vi "REV Sequence.vi"() -> ()   [LabVIEW 2026]
uses:
  <vilib>/REVLibDriver5/subvi/RevLibError.ctl
  <vilib>/REV Custom Controls/c_Spark_SparkModel.ctl
  <vilib>/REV Custom Controls/c_Spark_MotorType.ctl
  <vilib>/REV Custom Controls/c_Spark_ConfigParameter.ctl
  <vilib>/REV Custom Controls/c_Spark_ControlType.ctl
  236934de-075f-3feb-e829-b4f31b15ce3f.vi
  <vilib>/REVLibDriver5/REVLibDriver.lvlib
  lib/libREVLibDriver.so
  lvaddons/wpilib/1/MrcLib.lvlib
panel:
  out "function return 7":T1
  in  "Slide":dbl(slide) scale=-1.0..1.0
  out "function return 6":T1
  out "value out":u8
  out "function return 5":T1
  in  "idle":bool
  out "c_Spark_SparkModel":T2 items=["c_Spark_Unknown", "c_Spark_SparkFlex", "c_Spark_SparkMax"]
  out "function return 4":T1
  out "fwVersion out":T3
  in  "stop":bool
  out "function return 3":T1
  out "function return 2":T1
  out "function return":T1
  out "deviceId out":i32
  out "status out":T1
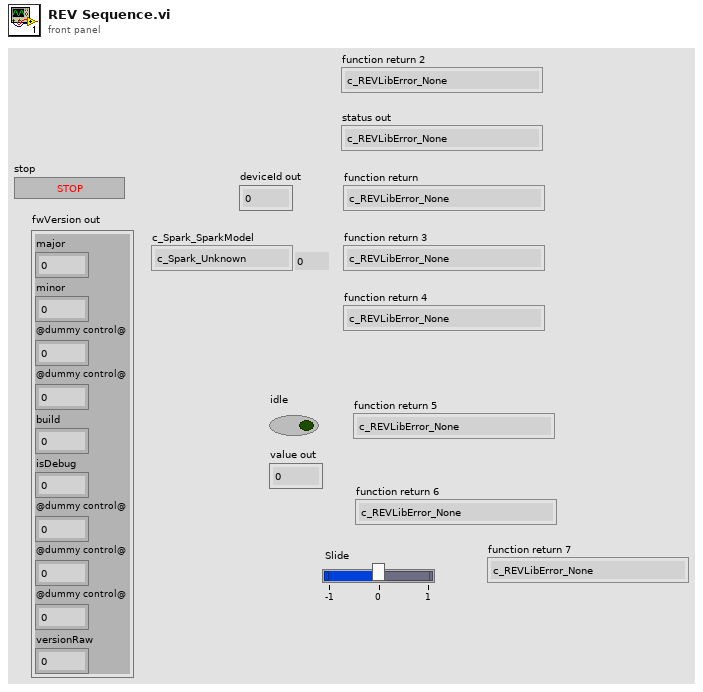
[diagram p1: front panel]
types:
  T1 = typedef "REVLibDriver.lvlib/RevLibError.ctl" = enum16{"c_REVLibError_None", "c_REVLibError_General", "c_REVLibError_CANTimeout", "c_REVLibError_NotImplemented", "c_REVLibError_HAL", "c_REVLibError_CantFindFirmware", "c_REVLibError_FirmwareTooOld", "c_REVLibError_FirmwareTooNew", "c_REVLibError_ParamInvalidID", "c_REVLibError_ParamMismatchType", "c_REVLibError_ParamAccessMode", "c_REVLibError_ParamInvalid", "c_REVLibError_ParamNotImplementedDeprecated", "c_REVLibError_FollowConfigMismatch", "c_REVLibError_Invalid", "c_REVLibError_SetpointOutOfRange", "c_REVLibError_Unknown", "c_REVLibError_CANDisconnected", "c_REVLibError_DuplicateCANId", "c_REVLibError_InvalidCANId", "c_REVLibError_SparkMaxDataPortAlreadyConfiguredDifferently", "c_REVLibError_SparkFlexBrushedWithoutDock", "c_REVLibError_InvalidBrushlessEncoderConfiguration", "c_REVLibError_FeedbackSensorIncompatibleWithDataPortConfig", "c_REVLibError_ParamInvalidChannel", "c_REVLibError_ParamInvalidValue", "c_REVLibError_CannotPersistParametersWhileEnabled", "c_REVLibError_NotReadyToReceiveCommand", "c_REVLibError_NumCodes"}
  T2 = typedef "REVLibDriver.lvlib/c_Spark_SparkModel.ctl" = u16
  T3 = cluster{"major":u8, "minor":u8, "@dummy control@":i8, "@dummy control@":i8, "build":u32, "isDebug":u8, "@dummy control@":i8, "@dummy control@":i8, "@dummy control@":i8, "versionRaw":u32}
  T4 = typedef "REVLibDriver.lvlib/c_Spark_ConfigParameter.ctl" = u16
  T5 = typedef "REVLibDriver.lvlib/c_Spark_MotorType.ctl" = enum16{"c_Spark_kMotorType_BRUSHED", "    c_Spark_kMotorType_BRUSHLESS", "    c_Spark_kNumMotorTypes"}
  T6 = typedef "REVLibDriver.lvlib/c_Spark_handle.ctl" = cluster{"Pointer":u64}
  T7 = typedef "REVLibDriver.lvlib/c_Spark_ControlType.ctl" = enum16{"c_Spark_kControlType_DUTY_CYCLE", "    c_Spark_kControlType_VELOCITY", "    c_Spark_kControlType_VOLTAGE", "    c_Spark_kControlType_POSITION", "    c_Spark_kControlType_CURRENT", "    c_Spark_kControlType_MAXMOTION_POSITION", "    c_Spark_kControlType_MAXMOTION_VELOCITY", "    c_Spark_kNumControlTypes"}
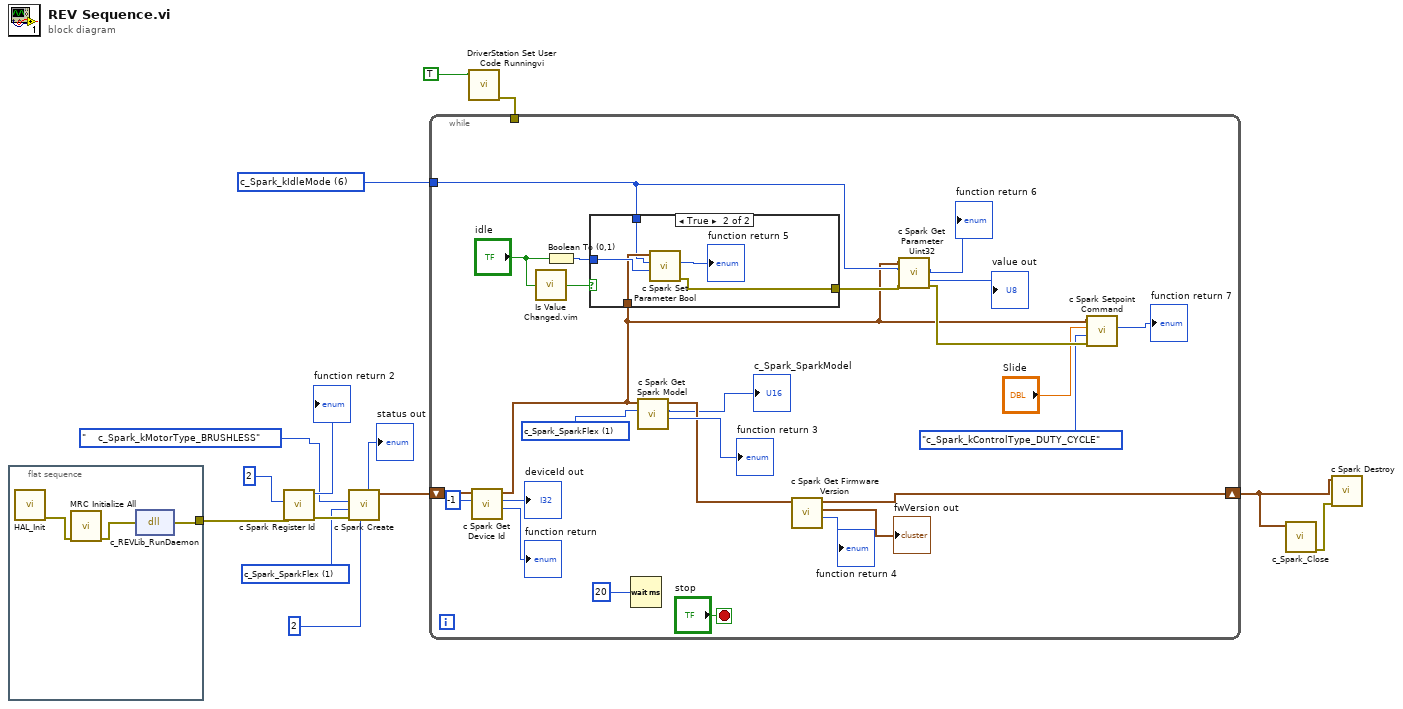
[diagram p0: block diagram]
diagram:
  w5 = T4 6 items=["   c_Spark_kCANID "=0, "    c_Spark_kInputMode "=1, "    c_Spark_kMotorType "=2, "    c_Spark_kCommutationAdvance "=3, "    c_Spark_kControlType "=5, "    c_Spark_kIdleMode "=6, "    c_Spark_kInputDeadband "=7, "    c_Spark_kClosedLoopControlSensor "=9, "    c_Spark_kPolePairs "=10, "    c_Spark_kCurrentChop "=11, "    c_Spark_kCurrentChopCycles "=12, "    c_Spark_kP_0 "=13, "    c_Spark_kI_0 "=14, "    c_Spark_kD_0 "=15, "    c_Spark_kV_0 "=16, "    c_Spark_kIZone_0 "=17, "    c_Spark_kDFilter_0 "=18, "    c_Spark_kOutputMin_0 "=19, "    c_Spark_kOutputMax_0 "=20, "    c_Spark_kP_1 "=21, "    c_Spark_kI_1 "=22, "    c_Spark_kD_1 "=23, "    c_Spark_kV_1 "=24, "    c_Spark_kIZone_1 "=25, "    c_Spark_kDFilter_1 "=26, "    c_Spark_kOutputMin_1 "=27, "    c_Spark_kOutputMax_1 "=28, "    c_Spark_kP_2 "=29, "    c_Spark_kI_2 "=30, "    c_Spark_kD_2 "=31, "    c_Spark_kV_2 "=32, "    c_Spark_kIZone_2 "=33, "    c_Spark_kDFilter_2 "=34, "    c_Spark_kOutputMin_2 "=35, "    c_Spark_kOutputMax_2 "=36, "    c_Spark_kP_3 "=37, "    c_Spark_kI_3 "=38, "    c_Spark_kD_3 "=39, "    c_Spark_kV_3 "=40, "    c_Spark_kIZone_3 "=41, "    c_Spark_kDFilter_3 "=42, "    c_Spark_kOutputMin_3 "=43, "    c_Spark_kOutputMax_3 "=44, "    c_Spark_kInverted "=45, "    c_Spark_kLimitSwitchFwdPolarity "=50, "    c_Spark_kLimitSwitchRevPolarity "=51, "    c_Spark_kHardLimitFwdEn "=52, "    c_Spark_kHardLimitRevEn "=53, "    c_Spark_kSoftLimitFwdEn "=54, "    c_Spark_kSoftLimitRevEn "=55, "    c_Spark_kOpenLoopRampRate "=56, "    c_Spark_kLegacyFollowerID "=57, "    c_Spark_kLegacyFollowerConfig "=58, "    c_Spark_kSmartCurrentStallLimit "=59, "    c_Spark_kSmartCurrentFreeLimit "=60, "    c_Spark_kSmartCurrentConfig "=61, "    c_Spark_kSmartCurrentReserved "=62, "    c_Spark_kMotorKv "=63, "    c_Spark_kEncoderCountsPerRev "=69, "    c_Spark_kEncoderAverageDepth "=70, "    c_Spark_kEncoderSampleDelta "=71, "    c_Spark_kEncoderInverted "=72, "    c_Spark_kVoltageCompensationMode "=74, "    c_Spark_kCompensatedNominalVoltage "=75, "    c_Spark_kIMaxAccum_0 "=96, "    c_Spark_kAllowedClosedLoopError_0 "=97, "    c_Spark_kIMaxAccum_1 "=100, "    c_Spark_kAllowedClosedLoopError_1 "=101, "    c_Spark_kIMaxAccum_2 "=104, "    c_Spark_kAllowedClosedLoopError_2 "=105, "    c_Spark_kIMaxAccum_3 "=108, "    c_Spark_kAllowedClosedLoopError_3 "=109, "    c_Spark_kClosedLoopRampRate "=114, "    c_Spark_kSoftLimitForward "=115, "    c_Spark_kSoftLimitReverse "=116, "    c_Spark_kAnalogAverageDepth "=121, "    c_Spark_kAnalogSensorMode "=122, "    c_Spark_kAnalogInverted "=123, "    c_Spark_kAnalogSampleDelta "=124, "    c_Spark_kCompatibilityPortConfig "=127, "    c_Spark_kAltEncoderCountsPerRev "=128, "    c_Spark_kAltEncoderAverageDepth "=129, "    c_Spark_kAltEncoderSampleDelta "=130, "    c_Spark_kAltEncoderInverted "=131, "    c_Spark_kNumParameters "=138, "    c_Spark_kDutyCycleInverted "=141, "    c_Spark_kDutyCycleAverageDepth "=143, "    c_Spark_kDutyCycleOffsetLegacy "=145, "    c_Spark_kDutyCycleRangeOffset "=146, "    c_Spark_kPositionPIDWrapEnable "=149, "    c_Spark_kDutyCycleSensorPrescaler "=153, "    c_Spark_kDutyCycleOffset "=154, "    c_Spark_kProductId "=155, "    c_Spark_kDeviceMajorVersion "=156, "    c_Spark_kDeviceMinorVersion "=157, "    c_Spark_kStatus0Period "=158, "    c_Spark_kStatus1Period "=159, "    c_Spark_kStatus2Period "=160, "    c_Spark_kStatus3Period "=161, "    c_Spark_kStatus4Period "=162, "    c_Spark_kStatus5Period "=163, "    c_Spark_kStatus6Period "=164, "    c_Spark_kStatus7Period "=165, "    c_Spark_kMAXMotionCruiseVelocity_0 "=166, "    c_Spark_kMAXMotionMaxAccel_0 "=167, "    c_Spark_kMAXMotionMaxJerk_0 "=168, "    c_Spark_kMAXMotionAllowedProfileError_0 "=169, "    c_Spark_kMAXMotionPositionMode_0 "=170, "    c_Spark_kMAXMotionCruiseVelocity_1 "=171, "    c_Spark_kMAXMotionMaxAccel_1 "=172, "    c_Spark_kMAXMotionMaxJerk_1 "=173, "    c_Spark_kMAXMotionAllowedProfileError_1 "=174, "    c_Spark_kMAXMotionPositionMode_1 "=175, "    c_Spark_kMAXMotionCruiseVelocity_2 "=176, "    c_Spark_kMAXMotionMaxAccel_2 "=177, "    c_Spark_kMAXMotionMaxJerk_2 "=178, "    c_Spark_kMAXMotionAllowedProfileError_2 "=179, "    c_Spark_kMAXMotionPositionMode_2 "=180, "    c_Spark_kMAXMotionCruiseVelocity_3 "=181, "    c_Spark_kMAXMotionMaxAccel_3 "=182, "    c_Spark_kMAXMotionMaxJerk_3 "=183, "    c_Spark_kMAXMotionAllowedProfileError_3 "=184, "    c_Spark_kMAXMotionPositionMode_3 "=185, "    c_Spark_kForceEnableStatus_0 "=186, "    c_Spark_kForceEnableStatus_1 "=187, "    c_Spark_kForceEnableStatus_2 "=188, "    c_Spark_kForceEnableStatus_3 "=189, "    c_Spark_kForceEnableStatus_4 "=190, "    c_Spark_kForceEnableStatus_5 "=191, "    c_Spark_kForceEnableStatus_6 "=192, "    c_Spark_kForceEnableStatus_7 "=193, "    c_Spark_kFollowerModeLeaderId "=194, "    c_Spark_kFollowerModeIsInverted "=195, "    c_Spark_kDutyCycleEncoderStartPulseUs "=196, "    c_Spark_kDutyCycleEncoderEndPulseUs "=197, "    c_Spark_kParamTableVersion "=198, "    c_Spark_kStatus8Period "=199, "    c_Spark_kForceEnableStatus_8 "=200, "    c_Spark_kLimitSwitchPositionSensor "=201, "    c_Spark_kLimitSwitchFwdPosition "=202, "    c_Spark_kLimitSwitchRevPosition "=203, "    c_Spark_kS_0 "=204, "    c_Spark_kA_0 "=205, "    c_Spark_kG_0 "=206, "    c_Spark_kCos_0 "=207, "    c_Spark_kCosRatio_0 "=208, "    c_Spark_kS_1 "=209, "    c_Spark_kA_1 "=210, "    c_Spark_kG_1 "=211, "    c_Spark_kCos_1 "=212, "    c_Spark_kCosRatio_1 "=213, "    c_Spark_kS_2 "=214, "    c_Spark_kA_2 "=215, "    c_Spark_kG_2 "=216, "    c_Spark_kCos_2 "=217, "    c_Spark_kCosRatio_2 "=218, "    c_Spark_kS_3 "=219, "    c_Spark_kA_3 "=220, "    c_Spark_kG_3 "=221, "    c_Spark_kCos_3 "=222, "    c_Spark_kCosRatio_3 "=223, "    c_Spark_kStatus9Period "=224, "    c_Spark_kForceEnableStatus_9 "=225, "    c_Spark_kDetachedEncoderDeviceID "=226] ("paramID")
  w13 = T2 1 items=["c_Spark_SparkMax"=0, "c_Spark_SparkFlex"=1, "c_Spark_Unknown"=255] ("unconfirmedModel")
  n1 = flat-sequence {
    tunnel: [w17] -> w7
    frame #0 {
      n2 = call "HAL_Init.vi"() -> ("error out"=w15:errorcluster)  [unwired: 11 in]
      n3 = call <vilib>:"MRC Initialize All.vi"("error out 2"=w15) -> ("error out"=w16:errorcluster)  [unwired: 10 in]
      n4 = dll-call lib="home/systemcore/natinst/lib/libREVLibDriver.so" fn="c_REVLib_RunDaemon"(error in=w16) -> (error out=w17:errorcluster)  [unwired: 3 in, 1 out]
    }
  }
  n5 = call <vilib>:"c Spark Register Id.vi"("error in (no error)"=w7, "deviceId"=2) -> ("error out"=w14:errorcluster, "function return"=→"function return 2":T1)  [unwired: 8 in]
  n6 = call <vilib>:"c Spark Create.vi"("deviceId"=2, "error in (no error)"=w14, "unconfirmedModel"=w13, "type"=c_Spark_MotorType."    c_Spark_kMotorType_BRUSHLESS") -> ("handle"=w10:T6, "status out"=→"status out":T1)  [unwired: 5 in, 1 out]
  n7 = call <vilib>:"DriverStation Set User Code Runningvi.vi"("code ready for enable"=TRUE) -> ("error out"=w3:errorcluster)  [unwired: 10 in]
  n8 = while {
    shift-right: [w31] -> w2
    shift-left: w10 -> [w42]
    tunnel: w5 -> [w26]
    tunnel: w3 -> [_]
    stop <- "stop" stop-if-true
    w32 = T2 1 items=["c_Spark_Unknown", "c_Spark_SparkFlex", "c_Spark_SparkMax"] ("model")
    n9 = call <vilib>:"c Spark Get Device Id.vi"("deviceId"=-1, "handle"=w42) -> ("function return"=→"function return":T1, "deviceId out"=→"deviceId out":i32, "handle out"=w21:T6)  [unwired: 6 in, 1 out]
    n10 = call "Is Value Changed.vim"("value"="idle") -> ("changed or first call?"=w27:bool)
    n11 = Boolean To (0,1)(Boolean="idle") -> (0, 1=w29:i16)
    n12 = case shown="True" w27 {
      tunnel: w29 -> [_ w47]
      tunnel: w21 -> [_ w46]
      tunnel: w26 -> [_ w44]
      tunnel: [_ w43] -> w25
      frame False {
      }
      frame True {
        n13 = call <vilib>:"c Spark Set Parameter Bool.vi"("value"=w47, "paramID"=w44, "handle"=w46) -> ("error out"=w43:errorcluster, "function return"=→"function return 5":T1)  [unwired: 6 in, 1 out]
      }
    }
    n14 = Wait (ms)(milliseconds to wait=u32 20) -> ()  [unwired: 1 out]
    n15 = call <vilib>:"c Spark Get Spark Model.vi"("c_Spark_SparkModel"=w32, "handle"=w21) -> ("function return"=→"function return 3":T1, "c_Spark_SparkModel"=→"c_Spark_SparkModel":T2, "handle out"=w36:T6)  [unwired: 6 in, 1 out]
    n16 = call <vilib>:"c Spark Get Firmware Version.vi"("handle"=w36) -> ("function return"=→"function return 4":T1, "fwVersion out"=→"fwVersion out":T3, "handle out"=w31:T6)  [unwired: 7 in, 1 out]
    n17 = call <vilib>:"c Spark Get Parameter Uint32.vi"("error in (no error)"=w25, "paramID"=w26, "handle"=w21) -> ("error out"=w22:errorcluster, "value out"=→"value out":u32, "function return"=→"function return 6":T1)  [unwired: 5 in, 1 out]
    n18 = call <vilib>:"c Spark Setpoint Command.vi"("error in (no error)"=w22, "ctrl"=c_Spark_ControlType."c_Spark_kControlType_DUTY_CYCLE", "value"="Slide", "handle"=w21) -> ("function return"=→"function return 7":T1)  [unwired: 5 in, 2 out]
  }
  n19 = call <vilib>:"c_Spark_Close.vi"("handle"=w2) -> ("error out"=w1:errorcluster)  [unwired: 10 in]
  n20 = call <vilib>:"c Spark Destroy.vi"("error in (no error)"=w1, "handle"=w2) -> ()  [unwired: 8 in, 2 out]
